vi "New Button.vi"(8 "error in (no error)":errorcluster, 9 "arguments":string, 10 "content":string) -> (0 "error out":errorcluster, 3 "new reference":refnum<k24>)   [LabVIEW 2026, in "ToastNotification.lvlib" / "Toast Native.lvlib"]
doc: "Construct a native ToastButton from visible content and raw activation arguments. new reference is acquired by the caller and must be closed after it is added to the builder or after a later error. This VI does not show the button or register callbacks."
uses:
  Toast Native.lvlib
  C:/Users/loicw/Documents/LabVIEW/ToastNotifications/Sources/bins/Microsoft.Toolkit.Uwp.Notifications.dll
  bins/Microsoft.Toolkit.Uwp.Notifications.dll
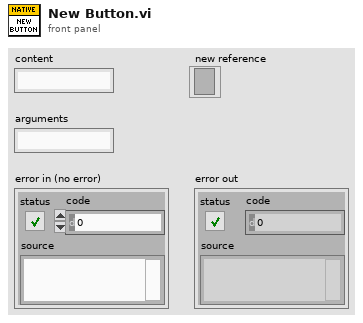
[diagram p1: front panel]
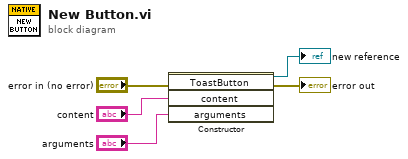
[diagram p0: block diagram]
diagram:
  n1 = constructor class="ToastButton"(error in="error in (no error)", "content"="content", "arguments"="arguments") -> (reference out=→"new reference":refnum<k24>, error out=→"error out":errorcluster)  [unwired: 2 in, 3 out]
